vi "Create LV RPC Method Name.vi"(1 "Proto Parser RPC Method Name in":string) -> (0 "LV RPC Method Name out":string)   [LabVIEW 2019, in "gRPC Template Creation Utility.lvlib"]
uses:
  gRPC Template Creation Utility.lvlib
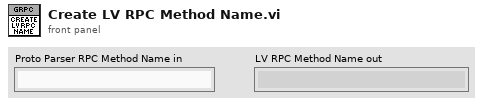
[diagram p1: front panel]
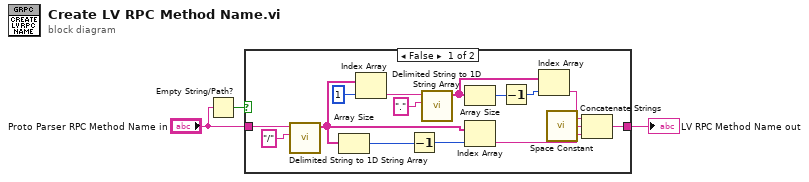
[diagram p0: block diagram]
diagram:
  n1 = Empty String/Path?(string/path="Proto Parser RPC Method Name in") -> (empty?=w3:bool)
  n2 = case shown="False" w3 {
    tunnel: [w5 w19] -> w1
    tunnel: "Proto Parser RPC Method Name in" -> [w17 w19]
    frame False {
      n3 = call <vilib>:"Delimited String to 1D String Array.vi"("delimiter"="/", "delimited string"=w17) -> ("string array"=w13:string[])  [unwired: 9 in]
      n4 = Array Size(array=w13) -> (size(s)=w12:i32)
      n5 = Index Array(array=w13, index=1) -> (element=w15:string)
      n6 = Decrement(x=w12) -> (x-1=w11:i32)
      n7 = call <vilib>:"Delimited String to 1D String Array.vi"("delimiter"=".", "delimited string"=w15) -> ("string array"=w8:string[])  [unwired: 9 in]
      n8 = Array Size(array=w8) -> (size(s)=w10:i32)
      n9 = Index Array(array=w13, index=w11) -> (element=w6:string)
      n10 = Decrement(x=w10) -> (x-1=w9:i32)
      n11 = Index Array(array=w8, index=w9) -> (element=w7:string)
      n12 = call <vilib>:"Space Constant.vi"() -> ("String"=w4:string)
      n13 = Concatenate Strings(w7, w4, w6) -> (w5:string)
    }
    frame True {
    }
  }
  "LV RPC Method Name out" <- w1
